vi "Frames_Create.vi"(8 "error in (no error)":errorcluster, 11 "capacity":i32=1756) -> (0 "error out":errorcluster, 3 "frames":T1 {"flags" format="%.0x"; "id" format="%.0x"})   [LabVIEW 2021, in "CANsub_API.lvlib" / "CANsub_Channel.lvclass"]
doc: "Makes a CANsub_Frames buffer for Read, owned by the caller (one per loop; keep it in a shift register). Capacity must be = the frames in one 4096-byte read (W1 max frames, 1756), else 5206. Setup/teardown only: do not call in a periodic loop (allocates, may block)."
uses:
  CANsub_Channel.lvclass
  CANsub_C.lvlib
  Typedefs/CANsub_Frames.ctl
  CANsub_API.lvlib
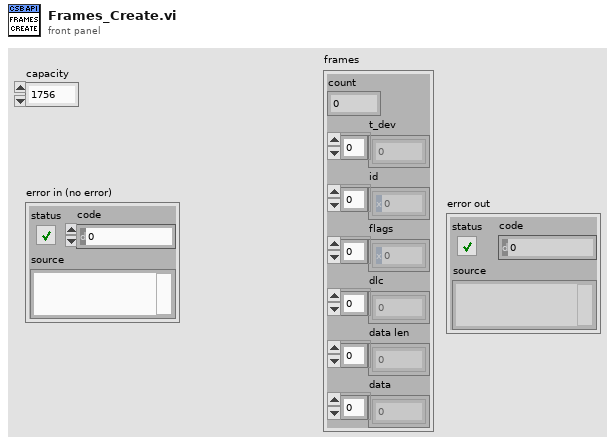
[diagram p1: front panel]
types:
  T1 = typedef "CANsub_API.lvlib/CANsub_Frames.ctl" = cluster{"count":i32, "t_dev":dbl[], "id":u32[], "flags":u16[], "dlc":u8[], "data len":u8[], "data":u8[]}
  T2 = typedef "CANsub_C.lvlib/C_Info.ctl" = cluster{"version":u32, "hdlc state size":i32, "ws state size":i32, "max frames (4096)":i32}
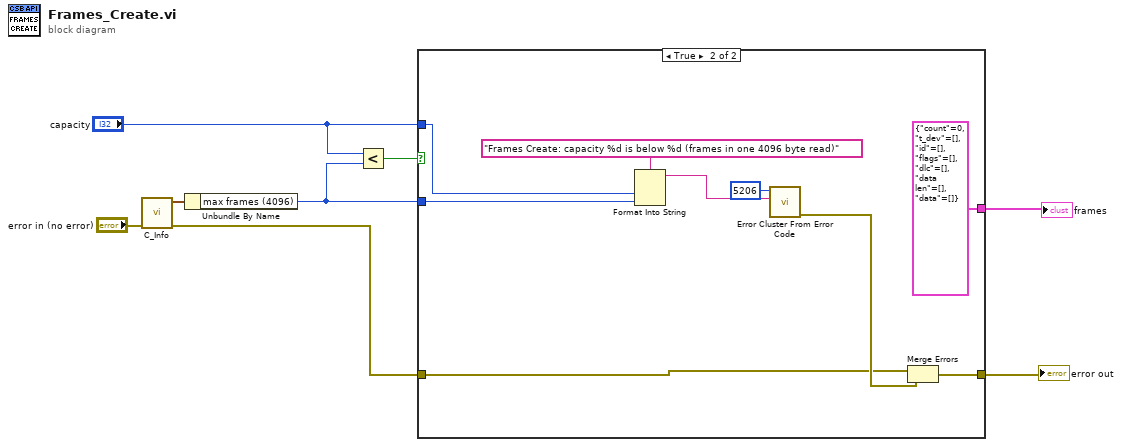
[diagram p0: block diagram]
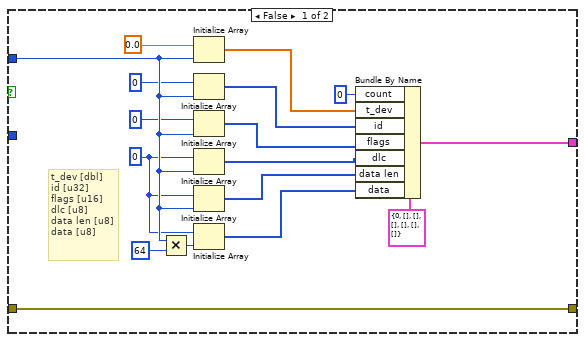
[diagram p2: hidden frame]
diagram:
  n1 = call "C_Info.vi"("error in (no error)"="error in (no error)") -> ("error out"=w2:errorcluster, "C_Info"=w7:T2)  [unwired: 9 in]
  n2 = Unbundle By Name(w7) -> ("max frames (4096)"=w1:i32)
  n3 = Less?(x="capacity", y=w1) -> (x < y?=w6:bool)
  n4 = case shown="True" w6 {
    tunnel: "capacity" -> [w24 w29]
    tunnel: [w10 T1 {"count"=0, "t_dev"=[], "id"=[], "flags"=[], "dlc"=[], "data len"=[], "data"=[]} ("frames")] -> w4
    tunnel: [w9 w32] -> w3
    tunnel: w2 -> [w9 w33]
    tunnel: w1 -> [_ w30]
    frame False {
      w22 = u8 0
      # "t_dev [dbl]\nid [u32]\nflags [u16]\ndlc [u8]\ndata len [u8]\ndata [u8]"
      n5 = Multiply(x=w24, y=64) -> (x*y=w25:i32)
      n6 = Initialize Array(0.0, w24) -> (w16:dbl[])
      n7 = Initialize Array(u32 0, w24) -> (w15:u32[])
      n8 = Initialize Array(u16 0, w24) -> (w14:u16[])
      n9 = Initialize Array(w22, w24) -> (w13:u8[])
      n10 = Initialize Array(w22, w24) -> (w12:u8[])
      n11 = Initialize Array(w22, w25) -> (w11:u8[])
      n12 = Bundle By Name(cluster=T1 {"count"=0, "t_dev"=[], "id"=[], "flags"=[], "dlc"=[], "data len"=[], "data"=[]} ("frames"), "count"=0, "t_dev"=w16, "id"=w15, "flags"=w14, "dlc"=w13, "data len"=w12, "data"=w11) -> (w10:T1)
    }
    frame True {
      n13 = Format Into String(format string="Frames Create: capacity %d is below %d (frames in one 4096 byte read)", w29, w30) -> (resulting string=w28:string)  [unwired: 2 in, 1 out]
      n14 = call <vilib>:"Error Cluster From Error Code.vi"("error message (\"\")"=w28, "error code (0)"=5206) -> ("error out"=w34:errorcluster)  [unwired: 7 in]
      n15 = Merge Errors(w33, w34) -> (w32:errorcluster)
    }
  }
  "error out" <- w3
  "frames" <- w4
